vi "UMLEditor Main.vi"(1 "StartProject":string, 3 "StartTarget":string) -> ()   [LabVIEW 2020] (continued)
                        n692 = call <resource>:"File_ApplicationPaths.vi"("PathName"=UMLEditor_StoredPathes."ClassBasePath" ("UMLPathes"), "Path In"=w1937, "Method (Get Path)"=w1936) -> ()  [unwired: 1 in, 16 out]
                      }
                    }
                  }
                  frame True {
                    n693 = property on="Target" class="Ring (strict)"("Strings []"=string[] [], "Value"=u16 0 ("icon")) -> ()  [unwired: 2 in, 2 out]
                  }
                }
                n694 = Bundle By Name(cluster=w1924, "Action"=w1904, "state"=UMLEditor_statesType."AnalyseViInStateDiagram") -> (w1923:T5)
              }
              frame "OpenUmlFile" {
                n695 = String To Path(string=w1946) -> (path=w1943:path)
                n696 = Bundle By Name(cluster=w1945, "state"=UMLEditor_statesType."Open", "file"=w1943) -> (w1944:T5)
              }
            }
          }
          event Application Instance Close? {
            n697 = event-data() -> ()  [unwired: 3 out]
            n698 = Bundle By Name(cluster=w1951, "state"=UMLEditor_statesType."Exit") -> (w1952:T5)
            n699 = event-data("Discard?"=TRUE) -> ()  [unwired: 1 in, 1 out]
          }
          event Key Down?; event type 5.0.x8000000b {
            (unwired) eventvkey."ASCII" ("VKey")
            n700 = event-data() -> ("Type"=w1958:T48, "Char"=w1966:i16, "VKey"=w1956:T47, "PlatMods"=w1965:T45)  [unwired: 3 out]
            n701 = Unbundle By Name(w1954) -> ("SelectedNodes"=w1960:refnum<class "AbstractNode.lvclass">[], "graphics"=w1957:refnum<class "Graphics.lvclass">)
            n702 = disable-structure shown="Disabled" {
              disable-tunnel: w1954 -> [w1969 w1971]
              disable-tunnel: [w1968 w1971] -> w1953
              frame Disabled {
                w1970 = FALSE ("Sync")
                n703 = Bundle By Name(cluster=w1969, "Sync"=w1970) -> (w1968:T5)
                n704 = local write "Sync"(w1970) -> ()
              }
              frame Enabled {
              }
            }
            n705 = Unbundle By Name(w1965) -> ("Ctrl"=w1955:bool, "Shift"=w1959:bool)
            n706 = case shown="\"Shift\"" w1956 {
              tunnel: w1956 -> [w1982 _ _ _]
              tunnel: w1953 -> [w1981 w2153 w2235 w2238]
              tunnel: [w1980 w2153 w2234 w2238] -> w1967
              tunnel: w1966 -> [w1979 _ _ _]
              tunnel: [w1977 w2152 w2233 w2237] -> w1964
              tunnel: w1963 -> [w1978 w2151 w2233 w2237]
              tunnel: w1962 -> [w1975 w2150 _ _]
              tunnel: w1954 -> [w1974 w2149 _ _]
              tunnel: w1961 -> [_ w2148 _ _]
              tunnel: w1960 -> [w1976 _ _ _]
              tunnel: w1959 -> [w1973 _ _ _]
              tunnel: w1958 -> [_ w2147 _ _]
              tunnel: w1957 -> [_ w2146 _ _]
              tunnel: w1955 -> [w1972 _ _ _]
              frame Default {
                n707 = case shown="False" w1972 {
                  tunnel: w1982 -> [w1992 _]
                  tunnel: w1981 -> [w1991 w2144]
                  tunnel: [w1990 w2144] -> w1980
                  tunnel: w1979 -> [w1989 _]
                  tunnel: w1978 -> [w1988 w2145]
                  tunnel: [w1987 w2145] -> w1977
                  tunnel: w1976 -> [w1986 _]
                  tunnel: w1975 -> [w1985 _]
                  tunnel: w1974 -> [w1984 _]
                  tunnel: w1973 -> [w1983 _]
                  frame False {
                    n708 = case shown="\"ASCII\"" w1992 {
                      selector: w1992 -> [_ _ _ w2073 _]
                      tunnel: w1991 -> [w2007 w2056 w2062 w2075 w2143]
                      tunnel: [w2010 w2055 w2061 w2076 w2143] -> w1990
                      tunnel: w1989 -> [w2005 _ _ _ _]
                      tunnel: w1988 -> [w1999 w2054 w2059 w2081 w2142]
                      tunnel: [w1998 w2054 w2059 w2080 w2142] -> w1987
                      tunnel: w1986 -> [_ _ _ w2079 _]
                      tunnel: w1985 -> [w1997 _ _ w2077 _]
                      tunnel: w1984 -> [_ _ _ w2074 _]
                      tunnel: w1983 -> [_ _ _ w2070 _]
                      frame "ASCII" {
                        n709 = Build Array(w2005) -> (w2004:i16[])
                        n710 = local read "SearchString"() -> (w2003:string)
                        n711 = Byte Array To String(unsigned byte array=w2004) -> (string=w2002:string)
                        n712 = Concatenate Strings(w2003, w2002) -> (w1996:string)
                        "SearchString" <- w1996
                        n713 = call <vilib>:"Trim Whitespace.vi"("string"=w1996) -> ("trimmed string"=w2001:string)  [unwired: 1 in]
                        n714 = Match Pattern(string=w1996, regular expression="^!") -> (after substring=w1993:string, offset past match=w1994:i32)  [unwired: 1 in, 2 out]
                        n715 = Equal?(x=w2005, y=i16 32) -> (x = y?=w2009:bool)
                        n716 = String Length(string=w2001) -> (length=w2000:i32)
                        n717 = Tick Count (ms)() -> (millisecond timer value=w2006:u32)
                        n718 = Bundle By Name(cluster=w2007, "KeyPressTime"=w2006) -> (w2008:T5)
                        n719 = case shown="Default" w2000 {
                          tunnel: [w2019 w2048] -> w2010
                          tunnel: w2009 -> [_ w2047]
                          tunnel: w2008 -> [w2018 w2046]
                          tunnel: w1999 -> [w2017 w2045]
                          tunnel: [w2016 w2045] -> w1998
                          tunnel: w1996 -> [w2015 _]
                          tunnel: w1997 -> [w2014 _]
                          tunnel: w1994 -> [w2013 _]
                          tunnel: w1993 -> [w2012 _]
                          frame Default {
                            n720 = case shown="-1" w2013 {
                              tunnel: [w2022 w2036] -> w2019
                              tunnel: w2018 -> [w2022 w2035]
                              tunnel: w2017 -> [w2021 w2034]
                              tunnel: [w2021 w2033] -> w2016
                              tunnel: w2015 -> [_ w2032]
                              tunnel: w2014 -> [_ w2031]
                              tunnel: w2012 -> [w2024 _]
                              frame 0, Default {
                                n721 = Match Pattern(string=w2024, regular expression="!$") -> (before substring=w2020:string, offset past match=w2023:i32)  [unwired: 1 in, 2 out]
                                n722 = case shown="0, Default" w2023 {
                                tunnel: w2020 -> [w2026 _]
                                frame 0, Default {
                                n723 = property on="PictureMenuEvent" class="Str"("Val(Sgnl)"=w2026) -> ()  [unwired: 2 in, 2 out]
                                n724 = local write "SearchString"("" ("SearchString")) -> ()
                                }
                                frame -1 {
                                }
                                }
                              }
                              frame -1 {
                                n725 = call-dynamic "FindNodeByName.vi"("reference"=w2031, "Name"=w2032, "error in (no error)"=w2034) -> ("node"=w2030:refnum<class "AbstractNode.lvclass">, "found"=w2029:bool, "error out"=w2033:errorcluster)  [unwired: 13 in, 1 out]
                                n726 = case shown="True" w2029 {
                                tunnel: [w2037 w2041] -> w2036
                                tunnel: w2035 -> [w2037 w2040]
                                tunnel: w2030 -> [_ w2039]
                                frame False {
                                }
                                frame True {
                                n727 = Build Array(w2039) -> (w2042:refnum<class "AbstractNode.lvclass">[])
                                n728 = Bundle By Name(cluster=w2040, "state"=UMLEditor_statesType."PanAndRepaint", "selected"=UMLEditor_tooltype."Node" ("selcted"), "SelectedNodes"=w2042, "newSelected"=TRUE) -> (w2041:T5)
                                }
                                }
                                n729 = property on="SearchString" class="Str"("Visible"=TRUE) -> ()  [unwired: 2 in, 2 out]
                              }
                            }
                          }
                          frame 0 {
                            n730 = case shown="False" w2047 {
                              tunnel: [w2049 w2053] -> w2048
                              tunnel: w2046 -> [w2049 w2052]
                              frame False {
                              }
                              frame True {
                                n731 = local write "GraphButtons"(T1."1" ("GraphButtons")) -> ()
                                n732 = Bundle By Name(cluster=w2052, "toolType"=UMLEditor_tooltype."None") -> (w2053:T5)
                              }
                            }
                          }
                        }
                      }
                      frame "Enter", "Return" {
                        n733 = Bundle By Name(cluster=w2056, "state"=UMLEditor_statesType."EditSelected") -> (w2055:T5)
                      }
                      frame "Delete" {
                        n734 = Bundle By Name(cluster=w2062, "state"=UMLEditor_statesType."RemoveSelected", "Don'tDeleteChildren"=FALSE) -> (w2061:T5)
                      }
                      frame "Up".."Right" {
                        w2078 = refnum<class "AbstractNode.lvclass">[] []
                        n735 = Unbundle By Name(w2074) -> ("gridSize"=w2068:dbl)
                        n736 = Select(t=5.0, s=w2070, f=1.0 ("t")) -> (s? t:f=w2069:dbl)
                        n737 = for {
                          tunnel: w2079 -> [w2104] mode=indexing
                          shift-right: [w2105] -> w2084
                          shift-left: w2078 -> [w2106]
                          n738 = call <resource>:"GetAllChildrenRecursive.vi"("reference"=w2104) -> ("children"=w2103:refnum<class "AbstractNode.lvclass">[])  [unwired: 1 in, 17 out]
                          n739 = Build Array (concatenate)(w2106, w2103) -> (w2105:refnum<class "AbstractNode.lvclass">[])
                        }
                        n740 = Multiply(x=w2069, y=w2068) -> (x*y=w2067:dbl)
                        n741 = case shown="\"Left\"" w2073 {
                          tunnel: w2067 -> [w2090 w2091 w2094 w2096]
                          tunnel: [0.0 ("t") 0.0 ("t") w2093 w2096] -> w2072
                          tunnel: [w2088 w2091 0.0 ("t") 0.0 ("t")] -> w2071
                          frame "Up" {
                            n742 = Negate(x=w2090) -> (-x=w2088:dbl)
                          }
                          frame "Down" {
                          }
                          frame "Left" {
                            n743 = Negate(x=w2094) -> (-x=w2093:dbl)
                          }
                          frame "Right", Default {
                          }
                        }
                        n744 = for {
                          tunnel: w2079 -> [w2131] mode=indexing
                          shift-right: [w2129] -> w2083
                          shift-left: w2081 -> [w2130]
                          tunnel: w2084 -> [w2118]
                          shift-right: [w2111] -> w2064
                          shift-left: w2078 -> [w2112]
                          tunnel: w2072 -> [w2109]
                          tunnel: w2071 -> [w2108]
                          w2120 = 0.0 ("t")
                          n745 = call-dynamic "getBounds.vi"("reference"=w2131, "error in (no error)"=w2130) -> ("reference out"=w2115:refnum<class "AbstractNode.lvclass">, "bounds"=w2128:T10, "error out"=w2116:errorcluster)  [unwired: 15 in]
                          n746 = Unbundle(w2128) -> ("x"=w2127:dbl, "y"=w2121:dbl)  [unwired: 2 out]
                          n747 = call-dynamic "getParent.vi"("reference"=w2115, "error in (no error)"=w2116) -> ("reference out"=w2113:refnum<class "AbstractNode.lvclass">, "parentNode"=w2110:refnum<class "AbstractNode.lvclass">, "ValidParent"=w2107:bool, "error out"=w2114:errorcluster)  [unwired: 13 in, 1 out]
                          n748 = Search 1D Array(1D array=w2118, element=w2115) -> (index of element=w2117:i32)  [unwired: 1 out]
                          n749 = Add(x=w2127, y=w2109) -> (x+y=w2126:dbl)
                          n750 = Add(x=w2121, y=w2108) -> (x+y=w2122:dbl)
                          n751 = Less Than 0?(x=w2126) -> (x < 0?=w2125:bool)
                          n752 = Less Than 0?(x=w2122) -> (x < 0?=w2123:bool)
                          n753 = case shown="True" w2107 {
                            tunnel: w2112 -> [w2132 w2135]
                            tunnel: [w2132 w2134] -> w2111
                            tunnel: w2110 -> [_ w2133]
                            frame False {
                            }
                            frame True {
                              n754 = Build Array (concatenate)(w2135, w2133) -> (w2134:refnum<class "AbstractNode.lvclass">[])
                            }
                          }
                          n755 = Select(t=w2120, s=w2125, f=w2109) -> (s? t:f=w2124:dbl)
                          n756 = Select(t=w2120, s=w2123, f=w2108) -> (s? t:f=w2119:dbl)
                          n757 = case shown="-1" w2117 {
                            tunnel: w2114 -> [w2136 w2141]
                            tunnel: [w2136 w2140] -> w2129
                            tunnel: w2124 -> [_ w2139]
                            tunnel: w2119 -> [_ w2138]
                            tunnel: w2113 -> [_ w2137]
                            frame 0, Default {
                            }
                            frame -1 {
                              n758 = call-dynamic "translate.vi"("reference"=w2137, "dx"=w2139, "dy"=w2138, "error in (no error)"=w2141) -> ("error out"=w2140:errorcluster)  [unwired: 14 in, 1 out]
                            }
                          }
                        }
                        n759 = Bundle By Name(cluster=w2075, "state"=UMLEditor_statesType."Repaint") -> (w2085:T5)
                        n760 = Array Size(array=w2064) -> (size(s)=w2063:i32)
                        n761 = case shown="Default" w2063 {
                          tunnel: w2083 -> [w2098 w2102]
                          tunnel: [w2098 w2101] -> w2082
                          tunnel: w2077 -> [_ w2100]
                          tunnel: w2064 -> [_ w2099]
                          frame Default {
                          }
                          frame 1.. {
                            n762 = call-dynamic "layout.vi"("reference"=w2100, "LayoutNodes(Empty=All)"=w2099, "error in (no error)"=w2102) -> ("error out"=w2101:errorcluster)  [unwired: 15 in, 1 out]
                          }
                        }
                        n763 = call <resource>:"UMLEditor setDiagramInfo.vi"("error in (no error)"=w2082, "localVariablesIn"=w2085, "action"=enum16{"Name/Dir", "Unsaved", "Saved"}."Unsaved") -> ("localVariablesOut"=w2076:T5, "error out"=w2080:errorcluster)  [unwired: 2 in, 13 out]
                      }
                      frame Default {
                      }
                    }
                  }
                  frame True {
                  }
                }
              }
              frame "Shift" {
                n764 = case shown="Default" w2147 {
                  tunnel: [w2154 w2160] -> w2152
                  tunnel: w2151 -> [w2154 w2159]
                  tunnel: w2150 -> [_ w2158]
                  tunnel: w2149 -> [_ w2157]
                  tunnel: w2148 -> [_ w2156]
                  tunnel: w2146 -> [_ w2155]
                  frame "Key Repeat?" {
                  }
                  frame Default {
                    n765 = case shown="\"ClassDiagramGraph\"" w2156 {
                      tunnel: [w2161 w2175] -> w2160
                      tunnel: w2159 -> [w2161 w2168]
                      tunnel: w2158 -> [_ w2174]
                      tunnel: w2157 -> [_ w2173]
                      tunnel: w2155 -> [_ w2169]
                      frame "None", Default {
                        # "Only supported in Class Diagram for now"
                      }
                      frame "ClassDiagramGraph" {
                        n766 = Unbundle By Name(w2173) -> ("zoom"=w2176:dbl, "offset"=w2178:T9)
                        n767 = property on="Picture" class="Pict"() -> ("Mouse"=w2172:T41)  [unwired: 2 in, 2 out]
                        n768 = Unbundle By Name(w2172) -> ("Mouse Position"=w2171:cluster{"X":i32, "Y":i32})
                        n769 = Add(x=w2178, y=w2171) -> (x+y=w2177:T9)
                        n770 = Divide(x=w2177, y=w2176) -> (x/y=w2162:T9)
                        n771 = call <resource>:"UMLEditor_FindObject.vi"("FindManyEdges(False)"=TRUE, "offset"=w2162, "error in"=w2168, "graphics"=w2169, "graph"=w2174) -> ("error out"=w2167:errorcluster, "NodeFound"=w2166:bool, "node"=w2179:refnum<class "AbstractNode.lvclass">, "edge"=w2170:refnum<class "AbstractEdge.lvclass">, "Edges"=w2163:refnum<class "AbstractEdge.lvclass">[], "EdgeFound"=w2165:bool)  [unwired: 1 in]
                        n772 = case shown="False" w2166 {
                          tunnel: [w2182 w2195] -> w2175
                          tunnel: w2179 -> [w2186 w2198]
                          tunnel: w2162 -> [w2185 w2197]
                          tunnel: w2167 -> [w2184 w2196]
                          tunnel: w2165 -> [_ w2194]
                          tunnel: w2170 -> [_ w2193]
                          tunnel: w2163 -> [_ w2192]
                          frame True {
                            n773 = call-dynamic "GetContextHelpInfo.vi"("reference"=w2186, "MousePos"=w2185, "error in (no error)"=w2184) -> ("ContextHelpInfoExist"=w2180:bool, "ContextHelpInfo"=w2181:variant, "error out"=w2183:errorcluster)  [unwired: 13 in, 1 out]
                            n774 = case shown="True" w2180 {
                              tunnel: w2183 -> [w2187 w2191]
                              tunnel: [w2187 w2190] -> w2182
                              tunnel: w2181 -> [_ w2189]
                              frame False {
                              }
                              frame True {
                                n775 = local write "Help"(TRUE ("Help")) -> ()
                                n776 = call <resource>:"ContextHelp_SendMessageToPopUp.vi"("PopUpMessage"=w2189, "error in (no error)"=w2191) -> ("error out"=w2190:errorcluster)  [unwired: 1 in, 16 out]
                              }
                            }
                          }
                          frame False {
                            n777 = case shown="True" w2194 {
                              tunnel: w2198 -> [_ _]
                              tunnel: w2197 -> [_ w2208]
                              tunnel: w2196 -> [w2199 w2211]
                              tunnel: [w2199 w2212] -> w2195
                              tunnel: w2193 -> [_ w2209]
                              tunnel: w2192 -> [_ w2207]
                              frame False {
                              }
                              frame True {
                                w2204 = cluster{string, "empty picture":picture, string} {"Dependencies", "empty picture"=bytes[0], ""}
                                n778 = for {
                                tunnel: w2209 -> [_]
                                tunnel: w2208 -> [w2217]
                                shift-right: [w2218] -> w2210
                                shift-left: w2211 -> [w2219]
                                tunnel: w2207 -> [w2216] mode=indexing
                                tunnel: w2204 -> [_]
                                shift-right: [w2213] -> w2202
                                shift-left: string[] [] -> [w2215]
                                n779 = call-dynamic "GetContextHelpInfo.vi"("reference"=w2216, "MousePos"=w2217, "error in (no error)"=w2219) -> ("Rows"=w2214:string[], "error out"=w2218:errorcluster)  [unwired: 12 in, 3 out]
                                n780 = for {
                                shift-right: [w2223] -> w2213
                                shift-left: w2215 -> [w2222]
                                tunnel: w2214 -> [w2221] mode=indexing
                                n781 = Search 1D Array(1D array=w2222, element=w2221) -> (index of element=w2220:i32)  [unwired: 1 in]
                                n782 = case shown="-1" w2220 {
                                tunnel: w2222 -> [w2224 w2227]
                                tunnel: w2221 -> [_ w2226]
                                tunnel: [w2224 w2225] -> w2223
                                frame Default {
                                }
                                frame -1 {
                                n783 = Build Array (concatenate)(w2227, w2226) -> (w2225:string[])
                                }
                                }
                                }
                                }
                                n784 = Concatenate Strings("<120>", w2202) -> (w2206:string)
                                n785 = Array Size(array=w2202) -> (size(s)=w2201:i32)
                                n786 = Bundle(cluster=w2204, w2206) -> (w2203:cluster{string, "empty picture":picture, string})  [unwired: 2 out]
                                n787 = case shown="1.." w2201 {
                                tunnel: w2210 -> [w2228 w2232]
                                tunnel: [w2228 w2231] -> w2212
                                tunnel: w2203 -> [_ w2230]
                                frame 0, Default {
                                }
                                frame 1.. {
                                n788 = local write "Help"(TRUE ("Help")) -> ()
                                n789 = call <resource>:"ContextHelp_SendMessageToPopUp.vi"("PopUpMessage"=w2230, "error in (no error)"=w2232) -> ("error out"=w2231:errorcluster)  [unwired: 1 in, 16 out]
                                }
                                }
                              }
                            }
                          }
                        }
                      }
                    }
                  }
                }
              }
              frame "F5" {
                n790 = Bundle By Name(cluster=w2235, "state"=UMLEditor_statesType."Repaint") -> (w2234:T5)
              }
              frame "Ctrl", "Alt" {
              }
            }
            n791 = event-data() -> ()  [unwired: 1 in, 6 out]
          }
          event Menu Selection (User) {
            n792 = event-data() -> ("MenuRef"=w2252:refnum<k9>, "ItemTag"=w2242:string)  [unwired: 1 out]
            n793 = Match Pattern(string=w2242, regular expression=":") -> (before substring=w2241:string, after substring=w2243:string)  [unwired: 1 in, 2 out]
            n794 = Match Pattern(string=w2241, regular expression="_[0-9]+$") -> (before substring=w2239:string)  [unwired: 1 in, 3 out]
            n795 = case shown="\"createScript\"" w2239 {
              selector: w2239 -> [_ _ _ _ _ _ _ _ _ w2368 _ _ _ _ w2402 w2409 _ _ _ _ _ w2545 w2554 w2569 w2585 w2608 _ _ _ _ _ _ _ _ _ _ _ _ _]
              tunnel: w2245 -> [w2254 w2289 w2291 w2299 w2315 w2326 w2336 w2342 w2348 w2365 w2381 w2383 w2389 w2395 w2404 w2411 w2414 w2451 w2473 w2481 w2509 w2547 w2557 w2571 w2589 w2611 w2621 w2626 w2628 w2632 w2636 w2642 w2646 w2650 w2654 w2657 w2660 w2678 w2687]
              tunnel: w2252 -> [_ _ _ _ _ _ _ _ _ w2362 _ _ _ _ _ _ _ _ _ _ _ _ w2562 w2575 _ _ _ _ _ _ _ _ _ _ _ _ _ _ _]
              tunnel: w2251 -> [w2260 w2288 w2290 w2296 w2320 w2331 w2333 w2337 w2352 w2359 w2380 w2385 w2391 w2397 w2403 w2413 w2416 w2447 w2477 w2479 w2501 w2549 w2561 w2574 w2588 w2600 w2619 w2623 w2627 w2629 w2633 w2640 w2644 w2649 w2652 w2656 w2661 w2674 w2688]
              tunnel: [w2260 w2287 w2290 w2292 w2316 w2327 w2333 w2337 w2351 w2370 w2380 w2385 w2391 w2397 w2403 w2413 w2415 w2450 w2477 w2479 w2491 w2549 w2555 w2566 w2587 w2596 w2619 w2623 w2627 w2629 w2633 w2640 w2644 w2649 w2652 w2655 w2661 w2663 w2688] -> w2250
              tunnel: [w2261 w2289 w2291 w2299 w2314 w2325 w2335 w2342 w2348 w2364 w2381 w2386 w2392 w2398 w2405 w2412 w2414 w2449 w2476 w2480 w2517 w2548 w2556 w2570 w2590 w2612 w2622 w2625 w2628 w2631 w2635 w2641 w2645 w2650 w2653 w2657 w2659 w2677 w2687] -> w2247
              tunnel: w2249 -> [w2259 _ _ _ w2319 w2330 _ _ _ _ _ _ _ _ _ _ _ _ _ _ _ _ _ _ _ w2595 _ _ _ _ _ _ _ _ _ _ _ w2666 _]
              tunnel: w2248 -> [_ _ _ _ _ _ _ _ _ _ _ _ _ _ _ _ _ _ _ _ _ _ _ _ _ w2594 _ _ _ _ _ w2639 _ _ _ _ _ _ _]
              tunnel: w2246 -> [_ _ _ _ w2312 w2323 _ _ _ _ _ _ _ _ _ _ _ _ _ _ _ _ _ _ _ _ _ _ _ _ _ _ _ _ _ _ _ _ _]
              tunnel: w2243 -> [_ _ _ _ _ _ _ _ _ _ _ _ _ _ _ _ _ _ _ _ w2500 _ _ _ _ _ _ _ _ _ _ _ _ _ _ _ _ _ _]
              tunnel: w2242 -> [w2256 _ _ _ _ _ _ _ _ _ _ _ _ _ _ _ _ _ _ _ _ _ _ _ _ _ _ _ _ _ _ _ _ _ _ _ _ _ _]
              frame Default {
                n796 = Unbundle By Name(w2254) -> ("selected"=w2253:T7, "selectedEdge"=w2258:refnum<class "AbstractEdge.lvclass">, "SelectedNodes"=w2257:refnum<class "AbstractNode.lvclass">[])
                n797 = call-dynamic "ExecuteToolMenuCommand.vi"("reference in"=w2259, "MenuItemTag"=w2256, "toolType"=w2253, "selectedEdge"=w2258, "SelectedNodes"=w2257, "error in (no error)"=w2260) -> ("Handled"=w2255:bool)  [unwired: 11 in, 2 out]
                n798 = case shown="False" w2255 {
                  tunnel: [w2268 w2284] -> w2261
                  tunnel: w2254 -> [w2264 w2285]
                  tunnel: w2256 -> [w2262 _]
                  frame False {
                    w2265 = FALSE ("Sync")
                    n799 = String To Path(string=w2262) -> (path=w2267:path)
                    n800 = File/Directory Info(path=w2267) -> (directory=w2270:bool, size=w2266:i64, error out=w2273:errorcluster)  [unwired: 1 in, 4 out]
                    n801 = local write "Sync"(w2265) -> ()
                    n802 = To Long Integer(number=w2266) -> (32bit integer=w2274:i32)
                    n803 = Unbundle By Name(w2273) -> ("status"=w2271:bool)
                    n804 = Greater Than 0?(x=w2274) -> (x > 0?=w2272:bool)
                    n805 = Bundle By Name(cluster=w2264, "Sync"=w2265) -> (w2263:T5)
                    n806 = Compound Arithmetic op=AND(invert w2270, w2272, invert w2271) -> (w2269:bool)
                    n807 = case shown="False" w2269 {
                      tunnel: w2263 -> [w2279 w2283]
                      tunnel: [w2279 w2282] -> w2268
                      tunnel: w2267 -> [w2278 w2280]
                      frame False {
                        n808 = Strip Path(path=w2278) -> (name=w2277:string)  [unwired: 1 out]
                        n809 = Format Into String(format string="File missing\nThis file could not be located.\n%s" ("message"), w2277) -> (resulting string=w2275:string)  [unwired: 2 in, 1 out]
                        n810 = One Button Dialog(message=w2275) -> ()  [unwired: 2 out]
                      }
                      frame True {
                        n811 = Bundle By Name(cluster=w2283, "state"=UMLEditor_statesType."Open", "file"=w2280) -> (w2282:T5)
                      }
                    }
                  }
                  frame True {
                    n812 = Bundle By Name(cluster=w2285, "state"=UMLEditor_statesType."Repaint") -> (w2284:T5)
                  }
                }
              }
              frame "About" {
                n813 = call <resource>:"OpenGDSLicense_ProductInfo.vi"("error in (no error)"=w2288) -> ("error out"=w2287:errorcluster)  [unwired: 18 in]
              }
              frame "APP_PROJECT_NEW" {
                n814 = invoke class="App" method="Project.NewWithPrompts"() -> ()  [unwired: 3 in, 3 out]
              }
              frame "OpenVI" {
                n815 = call "File Dialog2"("prompt"="Select VI to open", "error in"=w2296, "pattern (all files)"="*.vi") -> ("selected path"=w2294:path, "cancelled"=w2293:bool, "error out"=w2295:errorcluster)  [unwired: 4 in, 6 out]
                n816 = case shown="False" w2293 {
                  tunnel: w2295 -> [w2302 w2310]
                  tunnel: w2294 -> [w2301 _]
                  tunnel: [w2300 w2310] -> w2292
                  frame False {
                    n817 = call <resource>:"CommonVIs_UmlOpenVIRef.vi"("error in"=w2302) -> ("error out"=w2304:errorcluster, "AppRefOut"=w2303:refnum<vi>)  [unwired: 3 in, 6 out]
                    n818 = Open VI Reference(application reference (local)=w2303, vi path=w2301, error in (no error)=w2304) -> (vi reference=w2309:refnum<vi>, error out=w2305:errorcluster)  [unwired: 3 out]
                    n819 = property class="VI"(reference=w2309, error in=w2305, "Front Panel Window:Open"=TRUE) -> (reference out=w2307:refnum<vi>, error out=w2306:errorcluster)
                    n820 = Close Reference(reference=w2307, error in (no error)=w2306) -> (error out=w2300:errorcluster)
                  }
                  frame True {
                  }
                }
              }
              frame "Undo" {
                n821 = Unbundle By Name(w2312) -> ("graphics"=w2318:refnum<class "Graphics.lvclass">, "grid"=w2317:refnum<class "Grid.lvclass">)
                n822 = Unbundle By Name(w2312) -> ("menu"=w2311:refnum<k9>)
                n823 = call <resource>:"UndoEngine.vi"("Reference In"=w2319, "Action"=enum16{"TakeSnapshot", "Undo", "Redo"}."Undo", "graphics"=w2318, "grid"=w2317, "error in (no error)"=w2320, "menu"=w2311) -> ("error out"=w2316:errorcluster)  [unwired: 2 in, 11 out]
                n824 = Bundle By Name(cluster=w2315, "state"=UMLEditor_statesType."Repaint") -> (w2314:T5)
              }
              frame "Redo" {
                n825 = Unbundle By Name(w2323) -> ("graphics"=w2329:refnum<class "Graphics.lvclass">, "grid"=w2328:refnum<class "Grid.lvclass">)
                n826 = Unbundle By Name(w2323) -> ("menu"=w2322:refnum<k9>)
                n827 = call <resource>:"UndoEngine.vi"("Reference In"=w2330, "Action"=enum16{"TakeSnapshot", "Undo", "Redo"}."Redo", "graphics"=w2329, "grid"=w2328, "error in (no error)"=w2331, "menu"=w2322) -> ("error out"=w2327:errorcluster)  [unwired: 2 in, 11 out]
                n828 = Bundle By Name(cluster=w2326, "state"=UMLEditor_statesType."Repaint") -> (w2325:T5)
              }
              frame "EnterNewLicenceKey" {
                n829 = Bundle By Name(cluster=w2336, "state"=UMLEditor_statesType."CheckLicense") -> (w2335:T5)
              }
              frame "SendComments" {
                n830 = call <resource>:"UMLEditor CommentsDialog.vi"() -> ("nameOut"=w2340:string, "commentsOut"=w2339:string, "canceled"=w2338:bool, "error out"=w2341:errorcluster)  [unwired: 1 in, 15 out]
                n831 = case shown="True" w2338 {
                  tunnel: w2341 -> [w2346 w2347]
                  tunnel: w2340 -> [w2345 _]
                  tunnel: w2339 -> [w2344 _]
                  tunnel: [w2343 w2347] -> _
                  frame False {
                    n832 = call <resource>:"UMLEditor PostComment.vi"("name"=w2345, "comment"=w2344, "error in (no error)"=w2346) -> ("error out"=w2343:errorcluster)  [unwired: 16 out]
                  }
                  frame True {
                  }
                }
              }
              frame "Help_1" {
                n833 = local read "Help"() -> (w2350:bool)
                n834 = Not(x=w2350) -> (.not. x?=w2349:bool)
                n835 = local write "Help"(w2349) -> ()
                n836 = case shown="True" w2349 {
                  tunnel: [ContextHelp_HelpTexts."None(Hide)" ("HelpText") ContextHelp_HelpTexts."Default" ("HelpText")] -> w2353
                  frame False {
                  }
                  frame True {
                  }
                }
                n837 = call <resource>:"ContextHelp_HelpTexts.vi"("HelpText (enum or string)"=w2353) -> ("HelpOut"=w2354:T38)  [unwired: 18 out]
                n838 = call <resource>:"ContextHelp_SendMessageToPopUp.vi"("PopUpMessage"=w2354, "error in (no error)"=w2352) -> ("error out"=w2351:errorcluster)  [unwired: 1 in, 16 out]
              }
              frame "Help_Class Diagram", "Help_Sequence Diagram", "Help_State Diagram", "Help_Use Case Diagram" {
                n839 = local write "Help"("Help") -> ()
                n840 = Set Menu Item Info(6:FALSE ("ToolHelp"), 7:"Show Context Help for tools" ("item tag"), 8:w2359, 11:w2362) -> (0:w2367:errorcluster)  [unwired: 4 out]
                n841 = call <resource>:"ContextHelp_Memory.vi"("State"=FALSE ("ToolHelp"), "error in (no error)"=w2367, "Actio(GetStatus)n"=T23."SetToolHelp") -> ("error out"=w2360:errorcluster)  [unwired: 1 in, 15 out]
                n842 = case shown="True" "Help" {
                  tunnel: [ContextHelp_HelpTexts."None(Hide)" ("HelpText") w2375] -> w2371
                  tunnel: w2368 -> [_ w2374]
                  frame False {
                  }
                  frame True {
                    n843 = case shown="\"Help_Use Case Diagram\"" w2374 {
                      tunnel: [ContextHelp_HelpTexts."ClassDiagram_Help" ("HelpText") ContextHelp_HelpTexts."UseCaseDiagram_Help" ("HelpText") ContextHelp_HelpTexts."SequenceDiagram_Help" ("HelpText") ContextHelp_HelpTexts."StateDiagram_Help" ("HelpText")] -> w2375
                      frame "Help_Class Diagram", Default {
                      }
                      frame "Help_Use Case Diagram" {
                      }
                      frame "Help_Sequence Diagram" {
                      }
                      frame "Help_State Diagram" {
                      }
                    }
                  }
                }
                n844 = call <resource>:"ContextHelp_HelpTexts.vi"("HelpText (enum or string)"=w2371) -> ("HelpOut"=w2372:T38)  [unwired: 18 out]
                n845 = call <resource>:"ContextHelp_SendMessageToPopUp.vi"("PopUpMessage"=w2372, "error in (no error)"=w2360) -> ("error out"=w2370:errorcluster)  [unwired: 1 in, 16 out]
                n846 = Bundle By Name(cluster=w2365, "ToolHelp"=FALSE) -> (w2364:T5)
              }
              frame "GettingStarted" {
                n847 = call <resource>:"UMLEditor GettingStartedDialog.vi"() -> ()  [unwired: 1 out]
              }
              frame "Properties" {
                w2384 = FALSE ("Sync")
                n848 = Bundle By Name(cluster=w2383, "Sync"=w2384) -> (w2382:T5)
                n849 = local write "Sync"(w2384) -> ()
                n850 = Bundle By Name(cluster=w2382, "state"=UMLEditor_statesType."EditSelected") -> (w2386:T5)
              }
              frame "Class Reversed Engineering", "Class Reversed Engineering_2" {
                w2390 = FALSE ("Sync")
                n851 = Bundle By Name(cluster=w2389, "Sync"=w2390) -> (w2388:T5)
                n852 = local write "Sync"(w2390) -> ()
                n853 = Bundle By Name(cluster=w2388, "state"=UMLEditor_statesType."ClassReversedEngineering") -> (w2392:T5)
              }
              frame "State Reversed Engineering" {
                w2396 = FALSE ("Sync")
                n854 = Bundle By Name(cluster=w2395, "Sync"=w2396) -> (w2394:T5)
                n855 = local write "Sync"(w2396) -> ()
                n856 = Bundle By Name(cluster=w2394, "state"=UMLEditor_statesType."StateReversedEngineering") -> (w2398:T5)
              }
              frame "Delete", "Remove package only" {
                n857 = Equal?(x=w2402, y="Remove package only") -> (x = y?=w2400:bool)
                n858 = Bundle By Name(cluster=w2404, "state"=UMLEditor_statesType."RemoveSelected", "Don'tDeleteChildren"=w2400) -> (w2405:T5)
              }
              frame "Save", "Save As" {
                n859 = Equal?(x="Save As", y=w2409) -> (x = y?=w2407:bool)
                n860 = Bundle By Name(cluster=w2411, "state"=UMLEditor_statesType."Save", "saveAs"=w2407) -> (w2412:T5)
              }
              frame "Export to XMI" {
                (unwired) T49."new or existing file" ("select mode (2)")
                n861 = call <resource>:"UMLEditor getDiagramInfo.vi"("localVariables"=w2414, "error in (no error)"=w2416) -> ("graph"=w2417:refnum<class "Graph.lvclass">, "name"=w2423:string, "saveDir"=w2427:path, "error out"=w2418:errorcluster)  [unwired: 14 out]
                n862 = Build Path(base path=w2427, name or relative path=w2423) -> (appended path=w2424:path)
                n863 = call <vilib>:"Get File Extension.vi"("file"=w2424) -> ("filename without extension"=w2425:string)  [unwired: 1 in, 9 out]
                n864 = Concatenate Strings(w2425, ".xmi" ("string")) -> (w2428:string)
                n865 = File Dialog(6:"*.xmi" ("pattern"), 7:"Select file name" ("prompt"), 9:w2428, 11:w2427) -> (1:w2419:bool, 2:w2420:bool, 3:w2430:path)  [unwired: 1 in, 3 out]
                n866 = case shown="True" w2420 {
                  tunnel: [w2437 w2440] -> w2429
                  tunnel: w2419 -> [w2437 _]
                  tunnel: w2430 -> [w2438 w2439]
                  tunnel: [w2438 w2439] -> _
                  frame False {
                  }
                  frame True {
                    n867 = Two Button Dialog(message="This file already exists.\nDo you want to overwrite it?", 1:"No" ("F button name (\"Cancel\")"), 2:"Yes" ("T button name (\"OK\")")) -> (T button?=w2441:bool)
                    n868 = case shown="True" w2441 {
                      tunnel: w2439 -> [_ w2445]
                      frame False {
                      }
                      frame True {
                        n869 = Delete(path (use dialog)=w2445) -> ()  [unwired: 1 in, 6 out]
                      }
                    }
                    n870 = Not(x=w2441) -> (.not. x?=w2440:bool)
                  }
                }
                n871 = case shown="False" w2429 {
                  tunnel: w2417 -> [w2435 _]
                  tunnel: w2418 -> [w2434 w2436]
                  tunnel: w2430 -> [w2433 _]
                  tunnel: [w2431 w2436] -> w2415
                  frame False {
                    n872 = call-dynamic "saveGraph.vi"("reference"=w2435, "filePath"=w2433, "error in (no error)"=w2434, "ExportType(Normal)"=SaveTypes."XMI") -> ("error out"=w2431:errorcluster)  [unwired: 13 in, 2 out]
                  }
                  frame True {
                  }
                }
              }
              frame "Import from XMI" {
                n873 = call "File Dialog3"("prompt"="Select XMI file to import", "error in"=w2447, "pattern (all files)"="*.xm?", "pattern label"="XMI file") -> ("selected path"=w2448:path, "exists"=w2454:bool, "cancelled"=w2453:bool, "error out"=w2446:errorcluster)  [unwired: 8 in]
                n874 = Compound Arithmetic op=AND(w2454, invert w2453, invert w2446) -> (w2452:bool)
                n875 = case shown="False" w2452 {
                  tunnel: w2451 -> [w2458 w2464]
                  tunnel: w2447 -> [w2459 w2463]
                  tunnel: [w2459 w2463] -> w2450
                  tunnel: [w2458 w2465] -> w2449
                  tunnel: w2448 -> [_ w2462]
                  frame False {
                  }
                  frame True {
                    w2466 = FALSE ("Sync")
                    n876 = local write "Sync"(w2466) -> ()
                    n877 = Path To String(path=w2462) -> (string=w2461:string)
                    n878 = Bundle By Name(cluster=w2464, "selectedEdge"=refnum<class "AbstractEdge.lvclass"> refnum, "SelectedNodes"=refnum<class "AbstractNode.lvclass">[] [], "selected"=UMLEditor_tooltype."None" ("selcted"), "state"=UMLEditor_statesType."ClassReversedEngineering", "toolType"=UMLEditor_tooltype."None", "Sync"=w2466, "Action"=w2461, "XMI_Import"=TRUE ("Sync")) -> (w2465:T5)
                  }
                }
              }
              frame "Open" {
                w2474 = FALSE ("Sync")
                n879 = Bundle By Name(cluster=w2473, "Sync"=w2474) -> (w2472:T5)
                n880 = local write "Sync"(w2474) -> ()
                n881 = Bundle By Name(cluster=w2472, "state"=UMLEditor_statesType."Open") -> (w2476:T5)
              }
              frame "Close" {
                w2478 = FALSE ("Sync")
                n882 = Unbundle By Name(w2481) -> ("diagrams"=w2488:T8[])
                n883 = Array Size(array=w2488) -> (size(s)=w2487:i32)
                n884 = Greater Than 0?(x=w2487) -> (x > 0?=w2486:bool)
                n885 = Select(t=UMLEditor_statesType."Close" ("state"), s=w2486, f=UMLEditor_statesType."Idle" ("state")) -> (s? t:f=w2484:T6)
                n886 = local write "Sync"(w2478) -> ()
                n887 = Bundle By Name(cluster=w2481, "state"=w2484, "selected"=UMLEditor_tooltype."None" ("selcted"), "Sync"=w2478) -> (w2480:T5)
              }
              frame "Class Diagram", "New", "Sequence Diagram", "State Diagram", "Use Case Diagram" {
                w2507 = FALSE ("Sync")
                n888 = call <resource>:"CreateGraphFromName.vi"("GraphTypeToCreate"=w2500, "error in (no error)"=w2501) -> ("GraphCreated"=w2499:refnum<class "Graph.lvclass">, "error out"=w2498:errorcluster)  [unwired: 16 in]
                n889 = local write "GraphButtons"(T1."1" ("GraphButtons")) -> ()
                n890 = property on="GraphButtons" class="RadioBtnsControl (strict)"("Disabled"=u8 0) -> ()  [unwired: 2 in, 2 out]
                n891 = local write "Diagram"(0) -> ()
                n892 = property on="Picture" class="Pict"("Visible"=TRUE) -> ()  [unwired: 2 in, 2 out]
                n893 = call-dynamic "GetToolbarButtons.vi"("reference"=w2499, "error in (no error)"=w2498) -> ("reference out"=w2497:refnum<class "Graph.lvclass">, "AllToolbarButtons"=w2504:T36[], "error out"=w2506:errorcluster)  [unwired: 13 in, 2 out]
                n894 = Unbundle By Name(w2509) -> ("diagrams"=w2530:T8[])
                n895 = Unbundle By Name(w2509) -> ("menu"=w2508:refnum<k9>)
                n896 = call <resource>:"UpdateToolbar.vi"("ToolbarButtons"=w2504, "error in (no error)"=w2506) -> ("error out"=w2505:errorcluster)  [unwired: 17 in]
                n897 = for {
                  tunnel: w2530 -> [w2543] mode=indexing
                  tunnel: "Untitled %d" -> [w2541]
                  tunnel: [w2540] -> w2528 mode=indexing
                  n898 = Unbundle By Name(w2543) -> ("name"=w2542:string)
                  n899 = Scan From String(format string=w2541, input string=w2542) -> (output 1=w2540:i32)  [unwired: 2 in, 4 out]
                }
                n900 = call <resource>:"UndoEngine.vi"("Reference In"=w2497, "Action"=enum16{"TakeSnapshot", "Undo", "Redo"}."TakeSnapshot", "Reset"=TRUE, "error in (no error)"=w2505, "menu"=w2508) -> ("Reference Out"=w2493:refnum<class "Graph.lvclass">, "error out"=w2496:errorcluster)  [unwired: 3 in, 10 out]
                n901 = local read "Help"() -> (w2494:bool)
                n902 = Array Max & Min(array=w2528) -> (max value=w2527:i32)  [unwired: 3 out]
                n903 = case shown="True" w2494 {
                  tunnel: w2496 -> [w2532 w2538]
                  tunnel: [w2532 w2536] -> w2495
                  tunnel: w2493 -> [w2533 w2535]
                  tunnel: [w2533 w2534] -> w2489
                  frame False {
                  }
                  frame True {
                    n904 = call-dynamic "GetDiagramHelpText.vi"("reference in"=w2535, "error in (no error)"=w2538) -> ("reference out"=w2534:refnum<class "Graph.lvclass">, "HelpOut"=w2537:T38, "error out"=w2539:errorcluster)  [unwired: 15 in]
                    n905 = call <resource>:"ContextHelp_SendMessageToPopUp.vi"("PopUpMessage"=w2537, "error in (no error)"=w2539) -> ("error out"=w2536:errorcluster)  [unwired: 1 in, 16 out]
                  }
                }
                n906 = Increment(x=w2527) -> (x+1=w2525:i32)
                n907 = Format Into String(format string="Untitled %d", w2525) -> (resulting string=w2520:string)  [unwired: 2 in, 1 out]
                n908 = call <resource>:"UMLEditor addDiagram.vi"("graph"=w2489, "name"=w2520, "saveDir"=path "", "unsaved(False)"=FALSE, "error in (no error)"=w2495, "localVariablesIn"=w2509) -> ("localVariablesOut"=w2502:T5, "error out"=w2523:errorcluster)  [unwired: 1 in, 11 out]
                n909 = property on="Diagram" class="Ring (strict)"("Tip Strip"=w2520) -> ()  [unwired: 2 in, 2 out]
                n910 = Unbundle By Name(w2509) -> ("menu"=w2490:refnum<k9>)
                n911 = Bundle By Name(cluster=w2502, "selectedEdge"=refnum<class "AbstractEdge.lvclass"> refnum, "SelectedNodes"=refnum<class "AbstractNode.lvclass">[] [], "selected"=UMLEditor_tooltype."None" ("selcted"), "state"=UMLEditor_statesType."Repaint", "toolType"=UMLEditor_tooltype."None", "Sync"=w2507) -> (w2517:T5)
                n912 = call <resource>:"UMLEditor menuUpdates.vi"("menu"=w2490, "menuAction"=UMLEditor_MenuActionType."EnableSave", "error in (no error)"=w2523) -> ("error out"=w2492:errorcluster)  [unwired: 3 in, 13 out]
                n913 = local write "Sync"(w2507) -> ()
                n914 = call <resource>:"UMLEditor ToolsMenuUpdates.vi"("menu"=w2490, "Graph"=w2489, "error in (no error)"=w2492) -> ("error out"=w2491:errorcluster)  [unwired: 2 in, 14 out]
              }
              frame "Print", "jpg", "png" {
                n915 = case shown="\"Print\", Default" w2545 {
                  tunnel: [UMLEditor_ExportType."Printer" ("exportype") UMLEditor_ExportType."png" ("exportype") UMLEditor_ExportType."jpg" ("exportype")] -> w2544
                  frame "Print", Default {
                  }
                  frame "png" {
                  }
                  frame "jpg" {
                  }
                }
                n916 = Bundle By Name(cluster=w2547, "state"=UMLEditor_statesType."Export", "exportype"=w2544) -> (w2548:T5)
              }
              frame "Hide Grid" {
                n917 = Get Menu Item Info(7:w2554, 8:w2561, 11:w2562) -> (0:w2560:errorcluster, 3:w2553:refnum<k9>, 4:w2559:bool)  [unwired: 4 out]
                n918 = Not(x=w2559) -> (.not. x?=w2558:bool)
                n919 = Set Menu Item Info(6:w2558, 7:w2554, 8:w2560, 11:w2553) -> (0:w2555:errorcluster)  [unwired: 4 out]
                n920 = Bundle By Name(cluster=w2557, "state"=UMLEditor_statesType."Repaint", "hideGrid"=w2558) -> (w2556:T5)
              }
              frame "Show Context Help for tools" {
                n921 = Get Menu Item Info(7:w2569, 8:w2574, 11:w2575) -> (0:w2573:errorcluster, 3:w2568:refnum<k9>, 4:w2572:bool)  [unwired: 4 out]
                n922 = Not(x=w2572) -> (.not. x?=w2564:bool)
                n923 = Set Menu Item Info(6:w2564, 7:w2569, 8:w2573, 11:w2568) -> (0:w2567:errorcluster)  [unwired: 4 out]
                n924 = call <resource>:"ContextHelp_Memory.vi"("State"=w2564, "error in (no error)"=w2567, "Actio(GetStatus)n"=T23."SetToolHelp") -> ("error out"=w2566:errorcluster)  [unwired: 1 in, 15 out]
                n925 = Bundle By Name(cluster=w2571, "ToolHelp"=w2564) -> (w2570:T5)
              }
              frame "Zoom In", "Zoom Out" {
                w2580 = 1.5 ("x")
                n926 = Unbundle By Name(w2589) -> ("graphics"=w2591:refnum<class "Graphics.lvclass">, "zoom"=w2586:dbl)
                n927 = Equal?(x=w2585, y="Zoom In") -> (x = y?=w2582:bool)
                n928 = Square Root(x=w2580) -> ()  [unwired: 1 out]
                n929 = Multiply(x=w2586, y=w2580) -> (x*y=w2583:dbl)
                n930 = Divide(x=w2586, y=w2580) -> (x/y=w2581:dbl)
                n931 = Select(t=w2583, s=w2582, f=w2581) -> (s? t:f=w2577:dbl)
                n932 = In Range and Coerce(upper limit=5.0625, x=w2577, lower limit=0.197530864) -> (coerced(x)=w2576:dbl)  [unwired: 1 out]
                n933 = call <resource>:"scale.vi"("reference"=w2591, "scaleX"=w2576, "scaleY"=w2576, "error in (no error)"=w2588) -> ("error out"=w2587:errorcluster)  [unwired: 15 out]
                n934 = Bundle By Name(cluster=w2589, "zoom"=w2576, "state"=UMLEditor_statesType."Repaint") -> (w2590:T5)
              }
              frame "Larger Grid", "Smaller Grid" {
                n935 = Unbundle By Name(w2611) -> ("grid"=w2599:refnum<class "Grid.lvclass">, "gridSize"=w2610:dbl)
                n936 = Equal?(x=w2608, y="Larger Grid") -> (x = y?=w2605:bool)
                n937 = Square Root(x=2.0) -> (sqrt(x)=w2609:dbl)
                n938 = Multiply(x=w2610, y=w2609) -> (x*y=w2606:dbl)
                n939 = Divide(x=w2610, y=w2609) -> (x/y=w2604:dbl)
                n940 = call <resource>:"ForceUpdate.vi"("Set"=TRUE) -> ()  [unwired: 18 in, 1 out]
                n941 = Select(t=w2606, s=w2605, f=w2604) -> (s? t:f=w2603:dbl)
                n942 = In Range and Coerce(upper limit=100.0, x=w2603, lower limit=4.0) -> (coerced(x)=w2598:dbl)  [unwired: 1 out]
                n943 = call <resource>:"setGrid.vi"("reference"=w2599, "gridX"=w2598, "gridY"=w2598, "error in (no error)"=w2600) -> ("error out"=w2597:errorcluster)  [unwired: 15 out]
                n944 = case shown="Default" w2594 {
                  tunnel: w2597 -> [w2617 w2618]
                  tunnel: [w2616 w2618] -> w2596
                  tunnel: w2595 -> [w2615 _]
                  frame Default {
                    n945 = call-dynamic "layout.vi"("reference"=w2615, "error in (no error)"=w2617) -> ("error out"=w2616:errorcluster)  [unwired: 16 in, 1 out]
                  }
                  frame "None" {
                  }
                }
                n946 = Bundle By Name(cluster=w2611, "gridSize"=w2598, "state"=UMLEditor_statesType."Repaint") -> (w2612:T5)
              }
              frame "Exit" {
                n947 = Bundle By Name(cluster=w2621, "state"=UMLEditor_statesType."Exit") -> (w2622:T5)
              }
              frame "createScript" {
                n948 = Bundle By Name(cluster=w2626, "state"=UMLEditor_statesType."CreateScript") -> (w2625:T5)
              }
              frame "Open GOOP Wizard" {
                n949 = call <resource>:"UMLEditor SendMessageToWizard.vi"("error in (no error)"=w2627) -> ()  [unwired: 3 in, 16 out]
              }
              frame "Copy Selected Nodes" {
                n950 = Bundle By Name(cluster=w2632, "state"=UMLEditor_statesType."Copy") -> (w2631:T5)
              }
              frame "Paste Nodes" {
                n951 = Bundle By Name(cluster=w2636, "state"=UMLEditor_statesType."Paste") -> (w2635:T5)
              }
              frame "AutoPlace" {
                n952 = Not Equal?(x=T27 "", y=w2639) -> ()  [unwired: 1 out]
                n953 = Bundle By Name(cluster=w2642, "state"=UMLEditor_statesType."AutoPlace") -> (w2641:T5)
              }
              frame "Synchronize All" {
                n954 = Bundle By Name(cluster=w2646, "state"=UMLEditor_statesType."SyncAll") -> (w2645:T5)
              }
              frame "ToggleSync" {
                n955 = property on="Sync" class="Bool (strict)"() -> ("Value"=w2647:bool)  [unwired: 2 in, 2 out]
                n956 = Not(x=w2647) -> (.not. x?=w2648:bool)
                n957 = property on="Sync" class="Bool (strict)"("Val(Sgnl)"=w2648) -> ()  [unwired: 2 in, 2 out]
              }
              frame "StraightenAssociations" {
                n958 = Bundle By Name(cluster=w2654, "state"=UMLEditor_statesType."StraightenAssociation") -> (w2653:T5)
              }
              frame "Revision history" {
                n959 = call <resource>:"UMLEditor RevisionHistory.vi"("localVariables"=w2657, "error in (no error)"=w2656) -> ("error out"=w2655:errorcluster)  [unwired: 17 out]
              }
              frame "PlugInRev" {
                n960 = Bundle By Name(cluster=w2660, "state"=UMLEditor_statesType."PlugInReverseEngineering") -> (w2659:T5)
              }
              frame "Options" {
                n961 = call <resource>:"GetUndoOption.vi"("error in (no error)"=w2674) -> ("UndoSize"=w2671:i32, "error out"=w2673:errorcluster)  [unwired: 17 out]
                n962 = call <resource>:"UMLEditor_OptionsDialog.vi"("localVariables"=w2678, "error in (no error)"=w2673) -> ("error out"=w2672:errorcluster)  [unwired: 1 in, 16 out]
                n963 = call <resource>:"GetUndoOption.vi"("error in (no error)"=w2672) -> ("UndoSize"=w2665:i32, "error out"=w2669:errorcluster)  [unwired: 17 out]
                n964 = Unbundle By Name(w2678) -> ("menu"=w2667:refnum<k9>)
                n965 = Not Equal?(x=w2665, y=w2671) -> (x != y?=w2670:bool)
                n966 = case shown="True" w2670 {
                  tunnel: w2669 -> [w2679 w2686]
                  tunnel: [w2679 w2685] -> w2668
                  tunnel: w2667 -> [_ w2682]
                  tunnel: w2666 -> [_ w2681]
                  tunnel: w2665 -> [_ w2680]
                  frame False {
                  }
                  frame True {
                    n967 = call <resource>:"UndoEngine.vi"("Reference In"=w2681, "Action"=enum16{"TakeSnapshot", "Undo", "Redo"}."TakeSnapshot", "Reset"=TRUE, "error in (no error)"=w2686, "menu"=w2682, "UndoLevels(ignoredIfNotWired)"=w2680) -> ("error out"=w2685:errorcluster)  [unwired: 2 in, 11 out]
                  }
                }
                n968 = call <resource>:"UMLEditor AddToolsMenuItems.vi"("menu"=w2667, "GoopWizExists"=FALSE, "error in (no error)"=w2668) -> ("error out"=w2664:errorcluster)  [unwired: 1 in, 15 out]
                n969 = call <resource>:"GetSyncOption.vi"("error in (no error)"=w2664) -> ("SyncTime(s)"=w2662:i32, "error out"=w2663:errorcluster)  [unwired: 16 in, 1 out]
                n970 = Bundle By Name(cluster=w2678, "state"=UMLEditor_statesType."Repaint", "SyncTime"=w2662) -> (w2677:T5)
              }
              frame "ShowTips" {
                n971 = call <resource>:"ShowToolTips.vi"() -> ()  [unwired: 1 in, 19 out]
              }
            }
          }
          event Panel Close? {
            w2689 = FALSE ("Sync")
            n972 = event-data() -> ()  [unwired: 4 out]
            n973 = local write "Sync"(w2689) -> ()
            n974 = Bundle By Name(cluster=w2692, "state"=UMLEditor_statesType."Exit", "Sync"=w2689) -> (w2693:T5)
            n975 = event-data("Discard?"=TRUE) -> ()  [unwired: 1 in, 1 out]
          }
          event Panel Resize {
            w2695 = FALSE ("Sync")
            n976 = event-data() -> ()  [unwired: 9 out]
            n977 = local write "Sync"(w2695) -> ()
            n978 = Bundle By Name(cluster=w2698, "ResizePanelInProgress"=TRUE, "Sync"=w2695) -> (w2697:T5)
          }
          event Timeout {
            # "MouseDrag"
            n979 = event-data() -> ()  [unwired: 2 out]
            n980 = case shown="False" w2705 {
              tunnel: [w2715 w3042] -> w2700
              tunnel: w2704 -> [w2709 w3017]
              tunnel: w2703 -> [w2717 w3035]
              tunnel: [w2718 w3036] -> w2702
              tunnel: w2701 -> [w2716 w3014]
              frame False {
                n981 = property on="Picture" class="Pict"() -> ("Mouse"=w2713:T41)  [unwired: 2 in, 2 out]
                n982 = Unbundle By Name(w2713) -> ("Mouse Position"=w2708:cluster{"X":i32, "Y":i32}, "Mouse Modifiers.Shift Mod"=w2714:bool, "Mouse Modifiers.Menu Mod"=w2712:bool)
                n983 = Unbundle By Name(w2709) -> ("zoom"=w2706:dbl, "offset"=w2711:T9)
                n984 = Add(x=w2711, y=w2708) -> (x+y=w2710:T9)
                n985 = Divide(x=w2710, y=w2706) -> (x/y=w2707:T9)
                n986 = case shown="False" w2714 {
                  tunnel: w2717 -> [w2725 w2989]
                  tunnel: [w2724 w3000] -> w2718
                  tunnel: w2709 -> [w2722 w2990]
                  tunnel: w2716 -> [w2721 w2988]
                  tunnel: [w2726 w2990] -> w2715
                  tunnel: w2712 -> [w2723 _]
                  tunnel: w2707 -> [w2720 _]
                  tunnel: w2706 -> [w2719 _]
                  frame False {
                    n987 = Unbundle By Name(w2722) -> ("ResizePanelInProgress"=w2727:bool)
                    n988 = case shown="False" w2727 {
                      tunnel: w2722 -> [w2748 w2975]
                      tunnel: [w2738 w2973] -> w2726
                      tunnel: w2725 -> [w2752 w2971]
                      tunnel: [w2755 w2971] -> w2724
                      tunnel: w2722 -> [w2759 _]
                      tunnel: w2723 -> [w2756 _]
                      tunnel: w2722 -> [w2750 _]
                      tunnel: w2721 -> [w2753 _]
                      tunnel: w2720 -> [w2742 _]
                      tunnel: w2719 -> [w2735 _]
                      frame False {
                        # "Could generate Error when hibernating"
                        n989 = call <resource>:"GOOP_MouseFunctions.vi"("error in (no error)"=w2752) -> ("button info"=w2734:T50, "axis info"=w2751:T51)  [unwired: 8 in, 1 out]
                        n990 = Unbundle By Name(w2750) -> ("ObjectHotspots"=w2741:T15[])
                        n991 = Unbundle By Name(w2759) -> ("NodesBounds"=w2758:T10)
                        n992 = Unbundle By Name(w2750) -> ("KeyPressTime"=w2747:u32)
